vi "emur-char.vi"(11 "authority 2":u16(ring) items=["管理员", "操作员"]) -> (3 "字符串":string)   [LabVIEW 2018, in "login.lvlib"]
uses:
  login.lvlib
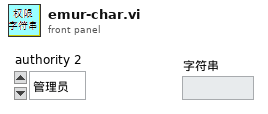
[diagram p1: front panel]
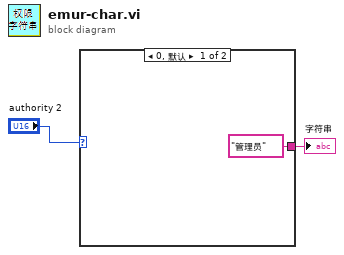
[diagram p0: block diagram]
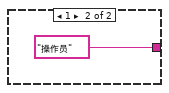
[diagram p2: hidden frame]
diagram:
  n1 = case shown="0, 默认" "authority 2" {
    tunnel: ["管理员" "操作员"] -> w1
    frame 0, Default {
    }
    frame 1 {
    }
  }
  "字符串" <- w1
